vi "SC Dialog.vi"(8 "Cancel text":string, 9 "message":string, 10 "window title":string, 11 "OK text":string="OK") -> (1 "OK?":bool)   [LabVIEW 2023]
doc: "A message dialog with a window title (LabVIEW's One and Two Button Dialogs have none, so their windows show as Untitled in a task bar): an OK button and, when Cancel text isn't empty, a Cancel button. OK? is true when the user clicks OK (or presses Enter); Cancel or closing the window gives false."
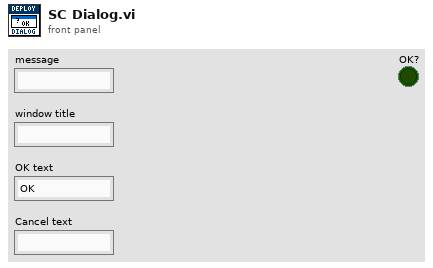
[diagram p1: front panel]
types:
  T1 = enum16{"Left Button", "Center Button", "Right Button", "Window Close"}
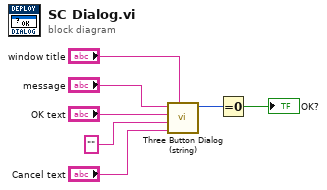
[diagram p0: block diagram]
diagram:
  n1 = call <vilib>:"Three Button Dialog (string).vi"("Window Title (\"\")"="window title", "Right Button Text (\"Cancel\")"="Cancel text", "Center Button Text (\"No\")"="", "Left Button Text (\"Yes\")"="OK text", "message"="message") -> ("Which Button?"=w2:T1)  [unwired: 6 in]
  n2 = Equal To 0?(x=w2) -> (x = 0?=→"OK?":bool)
